vi "包装工位流水码仅查验.vi"(11 "流水码编号":string) -> (0 "长度":i32, 1 "干检OK":i32, 2 "氦检OK":i32, 3 "可否包装":bool, 4 "没氦检":bool, 5 "烘干工位号":string)   [LabVIEW 2024]
panel:
  out "长度 2":i32
  out "没包装码":bool
  out "有客户码":bool
  out "结果字符串":string
  out "Rows Fetched":i32
  out "查重信息":string[][](array[string])
  out "error out":errorcluster
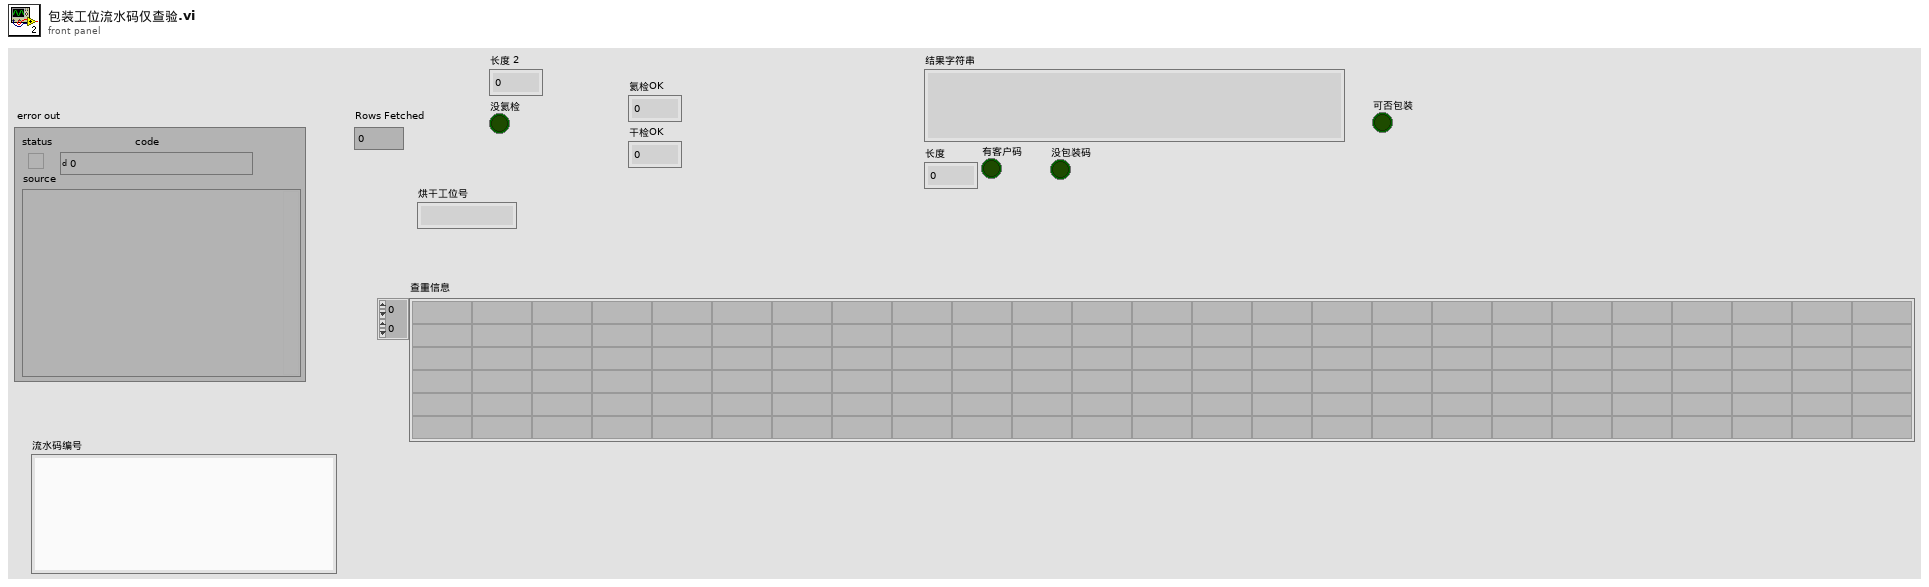
[diagram p1: front panel]
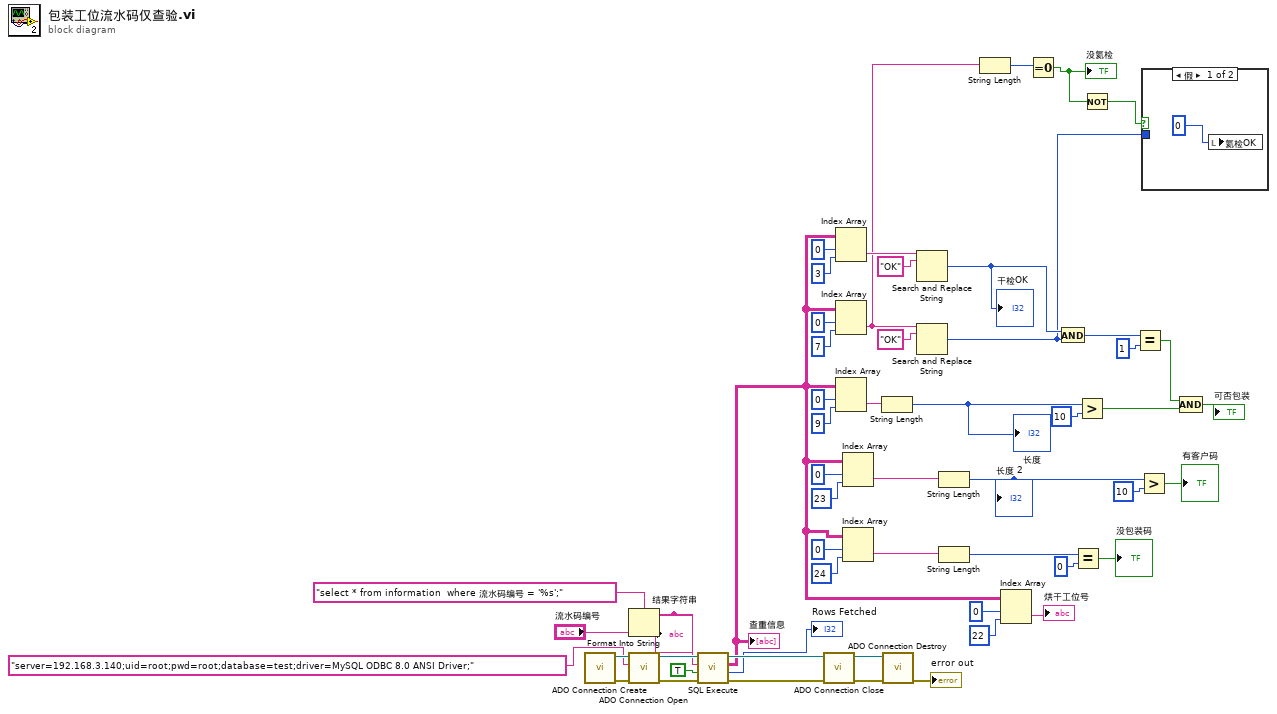
[diagram p0: block diagram]
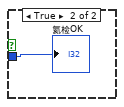
[diagram p2: hidden frame]
diagram:
  n1 = call "ADO Connection Create.vi"() -> ("error out"=w53:errorcluster, "ADODB._Connection Out"=w54:refnum<k7>)  [unwired: 10 in]
  n2 = Format Into String(format string="select * from information  where 流水码编号 = '%s';" ("Command Text"), "流水码编号") -> (resulting string=w14:string)  [unwired: 2 in, 1 out]
  "结果字符串" <- w14
  n3 = call "ADO Connection Open.vi"("error in (no error)"=w53, "ConnectionString"="server=192.168.3.140;uid=root;pwd=root;database=test;driver=MySQL ODBC 8.0 ANSI Driver;", "ADODB._Connection In"=w54) -> ("error out"=w51:errorcluster, "ADODB._Connection Out"=w52:refnum<k7>)  [unwired: 7 in]
  n4 = call "SQL Execute.vi"("error in (no error)"=w51, "Return Data (T)"=TRUE, "Command Text"=w14, "ADODB._Connection In"=w52) -> ("error out"=w49:errorcluster, "Rows Fetched"=→"Rows Fetched":i32, "Data"=w2:string[][], "ADODB._Connection Out"=w50:refnum<k7>)  [unwired: 4 in]
  "查重信息" <- w2
  n5 = call "ADO Connection Close.vi"("error in (no error)"=w49, "ADODB._Connection In"=w50) -> ("error out"=w47:errorcluster, "ADODB._Connection Out"=w48:refnum<k7>)  [unwired: 8 in]
  n6 = Index Array(array=w2, index (row)=0 ("禁用的索引 (行)"), index (col)=3 ("禁用的索引 (列)")) -> (element=w37:string)
  n7 = Index Array(array=w2, index (row)=0 ("禁用的索引 (行)"), index (col)=7 ("禁用的索引 (列)")) -> (element=w6:string)
  n8 = Index Array(array=w2, index (row)=0 ("禁用的索引 (行)"), index (col)=9 ("禁用的索引 (列)")) -> (element=w32:string)
  n9 = Index Array(array=w2, index (row)=0 ("禁用的索引 (行)"), index (col)=23 ("禁用的索引 (列)")) -> (element=w26:string)
  n10 = Index Array(array=w2, index (row)=0 ("禁用的索引 (行)"), index (col)=24 ("禁用的索引 (列)")) -> (element=w21:string)
  n11 = String Length(string=w32) -> (length=w12:i32)
  "长度" <- w12
  n12 = call "ADO Connection Destroy.vi"("error in (no error)"=w47, "ADODB._Connection In"=w48) -> ("error out"=→"error out":errorcluster)  [unwired: 9 in]
  n13 = Search and Replace String(input string=w37, search string="OK" ("搜索字符串")) -> (number of replacements=w35:i32)  [unwired: 6 in, 3 out]
  "干检OK" <- w35
  n14 = Search and Replace String(input string=w6, search string="OK" ("搜索字符串")) -> (number of replacements=w5:i32)  [unwired: 6 in, 3 out]
  n15 = String Length(string=w26) -> (length=w27:i32)
  "长度 2" <- w27
  n16 = String Length(string=w21) -> (length=w20:i32)
  n17 = String Length(string=w6) -> (length=w9:i32)
  n18 = Index Array(array=w2, index (row)=0 ("禁用的索引 (行)"), index (col)=22 ("禁用的索引 (列)")) -> (element=→"烘干工位号":string)
  n19 = Equal To 0?(x=w9) -> (x = 0?=w8:bool)
  "没氦检" <- w8
  n20 = And(x=w35, y=w5) -> (x .and. y?=w30:i32)
  n21 = Equal?(x=w20, y=0) -> (x = y?=→"没包装码":bool)
  n22 = Greater?(x=w12, y=10) -> (0:w17:bool)
  n23 = Not(x=w8) -> (.not. x?=w7:bool)
  n24 = Equal?(x=w30, y=1) -> (x = y?=w18:bool)
  n25 = Greater?(x=w27, y=10) -> (0:→"有客户码":bool)
  n26 = case shown="假" w7 {
    tunnel: w5 -> [_ w56]
    frame False {
      n27 = local write "氦检OK"(0 ("氦检OK")) -> ()
    }
    frame True {
      "氦检OK" <- w56
    }
  }
  n28 = Compound Arithmetic op=AND ("复合运算")(w18, w17) -> (→"可否包装":bool)
